vi "Running.vi"(8 "error in (no error)":errorcluster, 11 "CIFPlugin in":refnum<class "CAN_Reader_CANsub_Plugin.lvclass">) -> (0 "error out":errorcluster, 2 "Destroy":bool, 3 "CIFPlugin out":refnum<class "CAN_Reader_CANsub_Plugin.lvclass">)   [LabVIEW 2021, in "CAN_Reader_CANsub_Plugin.lvclass"]
uses:
  CAN_Reader_CANsub_Plugin.lvclass
  CAN_Reader_CANsub_Plugin.lvclass/CAN_Reader_CANsub_Plugin.ctl
  <vilib>/CIF Foundation/CIF Core/CIFCore/Class/CIFCorePlugin.lvclass
  <vilib>/CIF Foundation/CIF Core/CIFCore/Class/Typedef/Energized States.ctl
  C:/Program Files/National Instruments/LabVIEW 2021/vi.lib/CIF Foundation/CIF Core/CIFCore/Class/CIFCorePlugin.lvclass
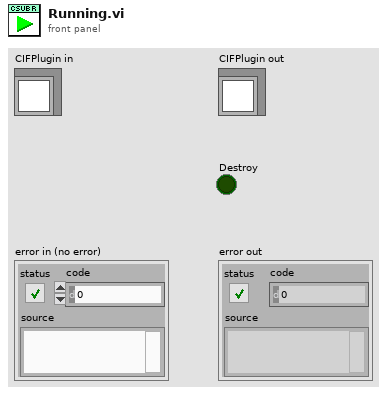
[diagram p1: front panel]
types:
  T1 = typedef "CIFCorePlugin.lvclass/Energized States.ctl" = enum8{"Listen", "Prepare", "Execute", "Housekeep", "Cleanup", "Destroy"}
  T2 = typedef "CIFCorePlugin.lvclass/Running State Logic.ctl" = enum8{"Execute", "Housekeep", "Cleanup", "Error", "Destroy"}
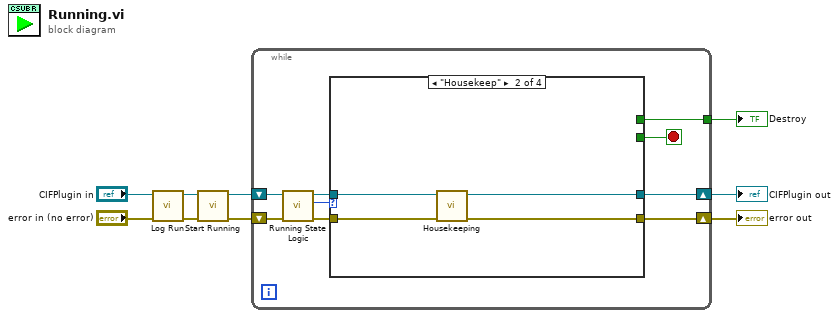
[diagram p0: block diagram]
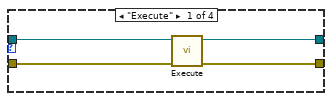
[diagram p2: hidden frame]
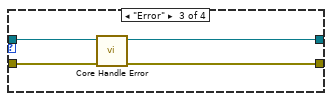
[diagram p3: hidden frame]
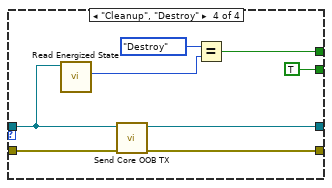
[diagram p4: hidden frame]
diagram:
  n1 = call <vilib>:"Log Run.vi"("error in (no error)"="error in (no error)", "CIFCorePlugin in"="CIFPlugin in") -> ("error out"=w7:errorcluster, "CIFCorePlugin out"=w6:refnum<class "CAN_Reader_CANsub_Plugin.lvclass">)  [unwired: 8 in]
  n2 = call <vilib>:"Start Running.vi"("error in (no error)"=w7, "CIFCorePlugin in"=w6) -> ("error out"=w8:errorcluster, "CIFCorePlugin out"=w9:refnum<class "CAN_Reader_CANsub_Plugin.lvclass">)  [unwired: 8 in]
  n3 = while {
    shift-right: [w13] -> w4
    shift-left: w9 -> [w18]
    shift-right: [w12] -> w3
    shift-left: w8 -> [w17]
    tunnel: [w10] -> w5
    stop <- w11 stop-if-true
    n4 = call <vilib>:"Running State Logic.vi"("error in (no error)"=w17, "CIFCorePlugin in"=w18) -> ("error out"=w14:errorcluster, "Running State Logic"=w16:T2, "CIFCorePlugin out"=w15:refnum<class "CAN_Reader_CANsub_Plugin.lvclass">)  [unwired: 7 in]
    n5 = case shown="\"Housekeep\"" w16 {
      tunnel: w15 -> [w22 w26 w30 w32]
      tunnel: w14 -> [w21 w25 w29 w37]
      tunnel: [w20 w24 w28 w36] -> w13
      tunnel: [w19 w23 w27 w35] -> w12
      tunnel: [_ _ _ TRUE] -> w11
      tunnel: [_ _ _ w33] -> w10
      frame "Execute" {
        n6 = call "Execute.vi"("error in (no error)"=w21, "CIFPlugin in"=w22) -> ("error out"=w19:errorcluster, "CIFPlugin out"=w20:refnum<class "CAN_Reader_CANsub_Plugin.lvclass">)  [unwired: 8 in]
      }
      frame "Housekeep" {
        n7 = call "Housekeeping.vi"("error in (no error)"=w25, "CIFPlugin in"=w26) -> ("error out"=w23:errorcluster, "CIFPlugin out"=w24:refnum<class "CAN_Reader_CANsub_Plugin.lvclass">)  [unwired: 8 in]
      }
      frame "Error" {
        n8 = call <vilib>:"Core Handle Error.vi"("error in (no error)"=w29, "CIFTemplateNode in"=w30) -> ("error out"=w27:errorcluster, "CIFTemplateNode out"=w28:refnum<class "CAN_Reader_CANsub_Plugin.lvclass">)  [unwired: 8 in]
      }
      frame "Cleanup", "Destroy" {
        n9 = call <vilib>:"Read Energized State.vi"("CIFCorePlugin in"=w32) -> ("Energized State"=w31:T1)  [unwired: 8 in, 2 out]
        n10 = call <vilib>:"Send Core OOB TX.vi"("error in (no error)"=w37, "CIFCorePlugin in"=w32) -> ("error out"=w35:errorcluster, "CIFCorePlugin out"=w36:refnum<class "CAN_Reader_CANsub_Plugin.lvclass">)  [unwired: 8 in]
        n11 = Equal?(x=Energized_States."Destroy", y=w31) -> (x = y?=w33:bool)
      }
    }
  }
  "error out" <- w3
  "Destroy" <- w5
  "CIFPlugin out" <- w4
